vi "Light_Update.vi"(0 "Comp":u8[][](array[numeric]), 1 "Old CX":i32=-100, 2 "Old CY":i32=-100, 3 "CX":i32, 5 "Lit":u8[][](array[numeric]), 7 "Dim":u8[][](array[numeric]), 9 "Dark":u8[][](array[numeric]), 11 "error in":errorcluster, 13 "CY":i32) -> (4 "Comp out":u8[][](array[numeric]), 6 "Rect":T1, 15 "error out":errorcluster)   [LabVIEW 2020, in "GH_Render.lvlib"]
doc: "Updates the composite picture of a dark room around Claude: every tile within 6 tiles of the old and the new centre comes from the lit (distance^2 <= 11), dim (<= 28) or dark picture. Old centre < -50 = only the new centre. Rect = the renewed tiles (left, top, right, bottom; right/bottom exclusive)."
uses:
  GH_Render.lvlib
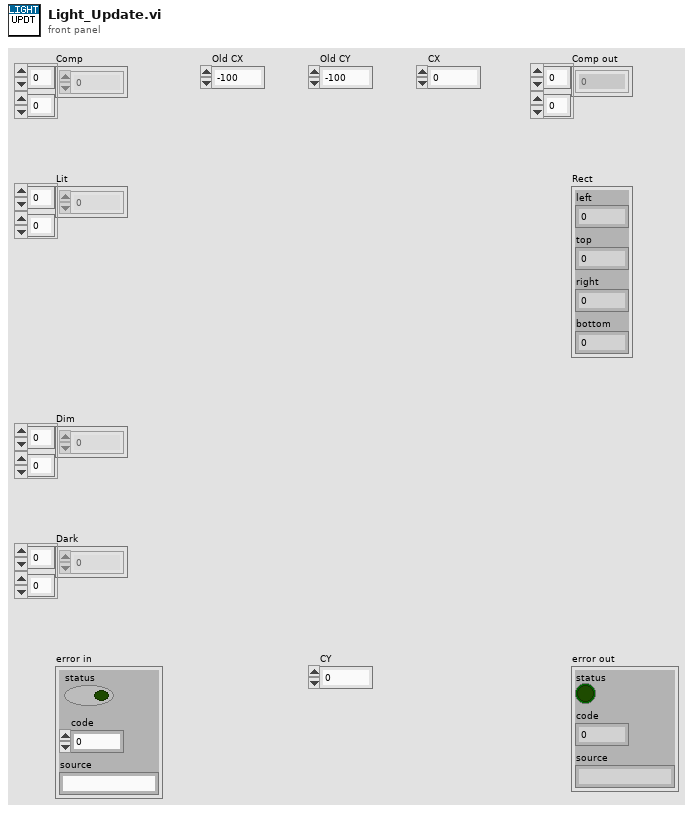
[diagram p1: front panel]
types:
  T1 = cluster{"left":i16, "top":i16, "right":i16, "bottom":i16}
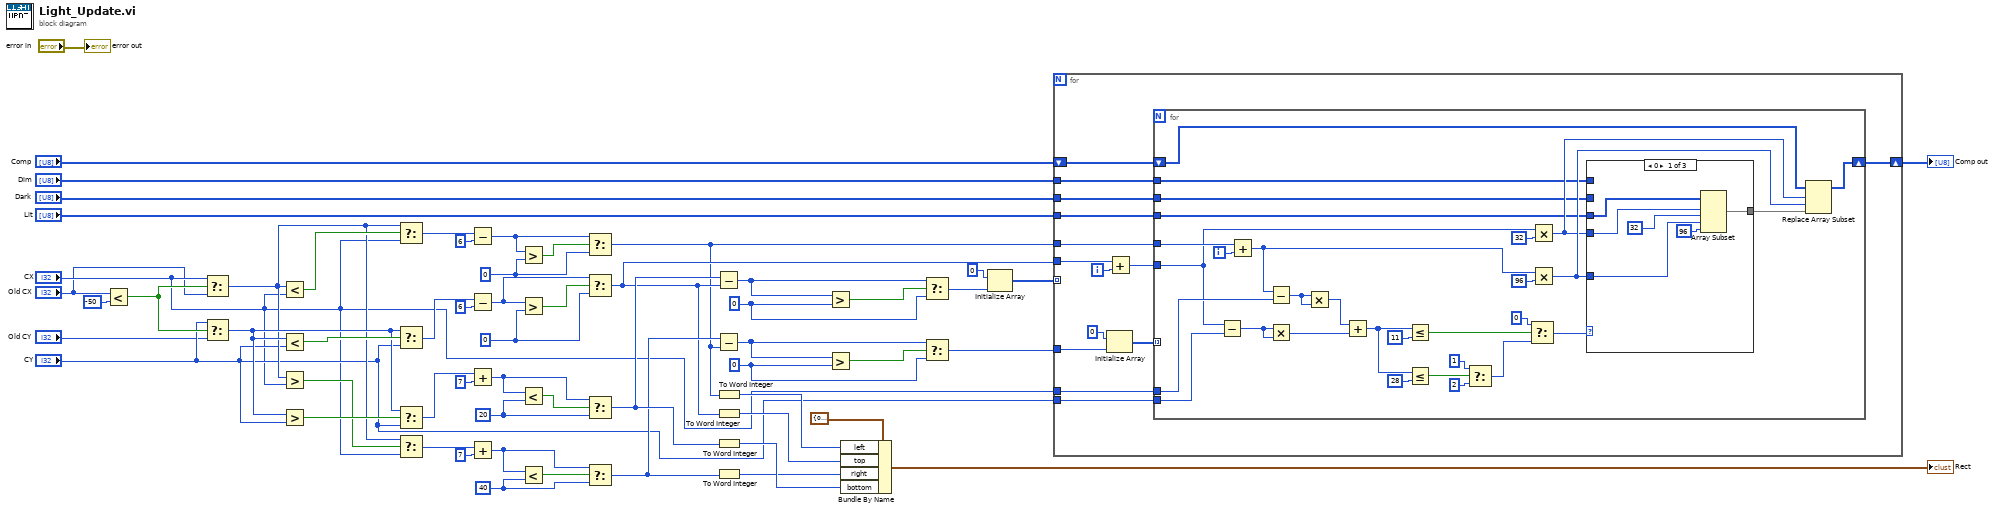
[diagram p0: block diagram]
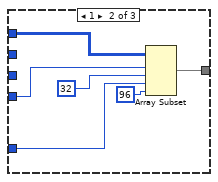
[diagram p2: hidden frame]
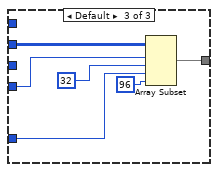
[diagram p3: hidden frame]
diagram:
  w47 = 0
  w43 = 0
  w39 = 20
  w32 = 40
  w25 = 0
  w18 = 0
  n1 = Less?(x="Old CX", y=-50) -> (x < y?=w11:bool)
  n2 = Select(t="CX", s=w11, f="Old CX") -> (s? t:f=w12:i32)
  n3 = Select(t="CY", s=w11, f="Old CY") -> (s? t:f=w13:i32)
  n4 = Less?(x=w12, y="CX") -> (x < y?=w14:bool)
  n5 = Less?(x=w13, y="CY") -> (x < y?=w21:bool)
  n6 = Greater?(x=w12, y="CX") -> (0:w28:bool)
  n7 = Greater?(x=w13, y="CY") -> (0:w35:bool)
  n8 = Select(t=w12, s=w14, f="CX") -> (s? t:f=w15:i32)
  n9 = Select(t=w13, s=w21, f="CY") -> (s? t:f=w22:i32)
  n10 = Select(t=w13, s=w35, f="CY") -> (s? t:f=w36:i32)
  n11 = Select(t=w12, s=w28, f="CX") -> (s? t:f=w29:i32)
  n12 = Subtract(x=w15, y=6) -> (x-y=w17:i32)
  n13 = Subtract(x=w22, y=6) -> (x-y=w24:i32)
  n14 = Add(x=w36, y=7) -> (x+y=w38:i32)
  n15 = Add(x=w29, y=7) -> (x+y=w31:i32)
  n16 = Greater?(x=w17, y=w18) -> (0:w19:bool)
  n17 = Greater?(x=w24, y=w25) -> (0:w26:bool)
  n18 = Less?(x=w38, y=w39) -> (x < y?=w40:bool)
  n19 = Less?(x=w31, y=w32) -> (x < y?=w33:bool)
  n20 = Select(t=w17, s=w19, f=w18) -> (s? t:f=w20:i32)
  n21 = Select(t=w24, s=w26, f=w25) -> (s? t:f=w27:i32)
  n22 = Select(t=w38, s=w40, f=w39) -> (s? t:f=w41:i32)
  n23 = Select(t=w31, s=w33, f=w32) -> (s? t:f=w34:i32)
  n24 = Subtract(x=w41, y=w27) -> (x-y=w42:i32)
  n25 = Subtract(x=w34, y=w20) -> (x-y=w46:i32)
  n26 = To Word Integer(number=w20) -> (16bit integer=w54:i16)
  n27 = To Word Integer(number=w27) -> (16bit integer=w55:i16)
  n28 = To Word Integer(number=w41) -> (16bit integer=w57:i16)
  n29 = To Word Integer(number=w34) -> (16bit integer=w56:i16)
  n30 = Greater?(x=w42, y=w43) -> (0:w44:bool)
  n31 = Greater?(x=w46, y=w47) -> (0:w48:bool)
  n32 = Bundle By Name(cluster=T1 {"left"=0, "top"=0, "right"=0, "bottom"=0}, "left"=w54, "top"=w55, "right"=w56, "bottom"=w57) -> (→"Rect":T1)
  n33 = Select(t=w42, s=w44, f=w43) -> (s? t:f=w45:i32)
  n34 = Select(t=w46, s=w48, f=w47) -> (s? t:f=w49:i32)
  n35 = Initialize Array(0, w45) -> (w51:i32[])
  n36 = for {
    tunnel: "Lit" -> [w60]
    tunnel: "Dim" -> [w61]
    tunnel: "Dark" -> [w62]
    tunnel: "CX" -> [w65]
    tunnel: "CY" -> [w66]
    shift-right: [w69] -> w52
    shift-left: "Comp" -> [w68]
    tunnel: w27 -> [w63]
    tunnel: w20 -> [w64]
    tunnel: w49 -> [w67]
    tunnel: w51 -> [_] mode=indexing
    i -> [w59]
    n37 = Initialize Array(0, w67) -> (w72:i32[])
    n38 = Add(x=w63, y=w59) -> (x+y=w70:i32)
    n39 = for {
      tunnel: w60 -> [w74]
      tunnel: w61 -> [w75]
      tunnel: w62 -> [w76]
      tunnel: w65 -> [w79]
      tunnel: w66 -> [w80]
      shift-right: [w82] -> w69
      shift-left: w68 -> [w81]
      tunnel: w64 -> [w78]
      tunnel: w70 -> [w77]
      tunnel: w72 -> [_] mode=indexing
      i -> [w73]
      n40 = Subtract(x=w77, y=w80) -> (x-y=w85:i32)
      n41 = Add(x=w78, y=w73) -> (x+y=w83:i32)
      n42 = Subtract(x=w83, y=w79) -> (x-y=w84:i32)
      n43 = Multiply(x=w85, y=w85) -> (x*y=w87:i32)
      n44 = Multiply(x=w84, y=w84) -> (x*y=w86:i32)
      n45 = Add(x=w86, y=w87) -> (x+y=w88:i32)
      n46 = Less Or Equal?(x=w88, y=11) -> (x <= y?=w90:bool)
      n47 = Less Or Equal?(x=w88, y=28) -> (x <= y?=w93:bool)
      n48 = Select(t=1, s=w93, f=2) -> (s? t:f=w96:i32)
      n49 = Select(t=0, s=w90, f=w96) -> (s? t:f=w97:i32)
      n50 = Multiply(x=w77, y=32) -> (x*y=w99:i32)
      n51 = Multiply(x=w83, y=96) -> (x*y=w101:i32)
      n52 = case shown="0" w97 {
        tunnel: w74 -> [w103 _ _]
        tunnel: w75 -> [_ w109 _]
        tunnel: w76 -> [_ _ w115]
        tunnel: w99 -> [w104 w110 w116]
        tunnel: w101 -> [w105 w111 w117]
        tunnel: [w108 w114 w120] -> w102
        frame 0 {
          n53 = Array Subset(array=w103, index (row)=w104, length (row)=32, index (col)=w105, length (col)=96) -> (w108:u8[][])
        }
        frame 1 {
          n54 = Array Subset(array=w109, index (row)=w110, length (row)=32, index (col)=w111, length (col)=96) -> (w114:u8[][])
        }
        frame Default {
          n55 = Array Subset(array=w115, index (row)=w116, length (row)=32, index (col)=w117, length (col)=96) -> (w120:u8[][])
        }
      }
      n56 = Replace Array Subset(array=w81, new element=w102, index (row)=w99, index (col)=w101) -> (w82:u8[][])
    }
  }
  "Comp out" <- w52
  "error out" <- "error in"
